vi "Verify Type.vi"(8 "error in (no error)":errorcluster, 11 "CIF_CIPC_Universal in":refnum<class "CIF_Iceoryx_Universal.lvclass">) -> (0 "error out":errorcluster, 3 "CIF_CIPC_Universal out":refnum<class "CIF_Iceoryx_Universal.lvclass">)   [LabVIEW 2021, in "CIF_Iceoryx_Universal.lvclass"]
uses:
  CIF_Iceoryx_Universal.lvclass
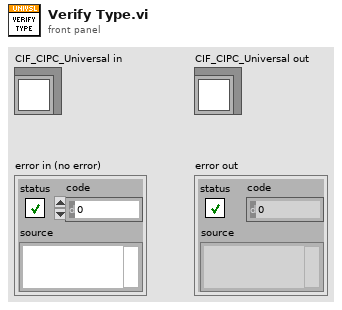
[diagram p1: front panel]
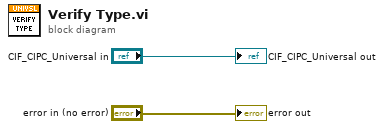
[diagram p0: block diagram]
diagram:
  "error out" <- "error in (no error)"
  "CIF_CIPC_Universal out" <- "CIF_CIPC_Universal in"
